vi "Equal Type Comparison.vi"(6 "verbose? (F)":bool, 8 "error in (no error)":errorcluster, 9 "Actual":variant, 10 "Expected":variant) -> (0 "error out":errorcluster, 2 "Equal Types?":bool, 3 "Verbose output":string)   [LabVIEW 2013, in "Caraya.lvlib" / "Assert.lvclass"]
uses:
  classes/Assert/Assert.lvclass
  <vilib>/Utility/VariantDataType/Type.ctl
  <vilib>/Utility/VariantDataType/VariantType.lvlib
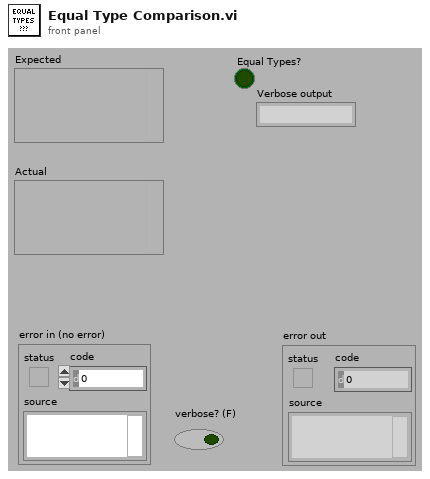
[diagram p1: front panel]
types:
  T1 = typedef "VariantType.lvlib/Type.ctl" = enum8{"Invalid Type", "Void", "I8", "I16", "I32", "I64", "U8", "U16", "U32", "U64", "Single Float", "Double Float", "Extended Float", "Single Complex", "Double Complex", "Extended Complex", "Enum U8", "Enum U16", "Enum U32", "Enum U64", "Single Float With Unit", "Double Float With Unit", "Extended Float With Unit", "Single Complex with Unit", "Double Complex with Unit", "Extended Complex with Unit", "Boolean", "String", "Path", "Picture", "Tag", "Array", "Cluster", "Variant", "LV Variant", "Waveform", "Timestamp", "Digital Waveform", "Digital Data", "ExpressData", "Refnum", "External Data", "VI", "Poly VI", "LabVIEW Class Instance", "Fixed Point"}
  T2 = typedef "VariantType.lvlib/RefnumType.ctl" = enum16{"NotARefnum", "UnknownRefnum", "Generic", "Datalog", "ByteStream", "Device", "Occurence", "TCPNetConnection", "Auto", "Menu", "Imaq", "Hardware", "DataSocket", "Visa", "IVI", "UDPNetConnection", "Notifier", "Queue", "Irda", "EventReg", "DotNet", "UserEvent", "Callback", "UNUSED_EMPTY_POSITION", "BlueToothNetConnection", "LVObjApp", "LVObjVI", "LVObjUnknown", "GenericClass", "UserDefinedRefnumTag", "DataValue", "RT FIFO", "TDMS File"}
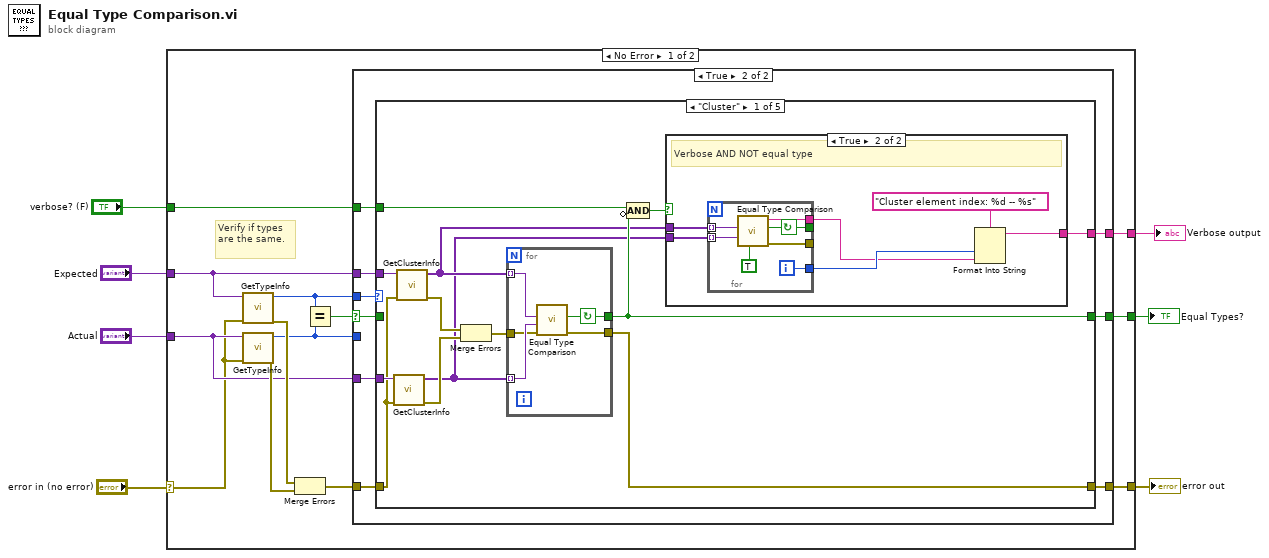
[diagram p0: block diagram]
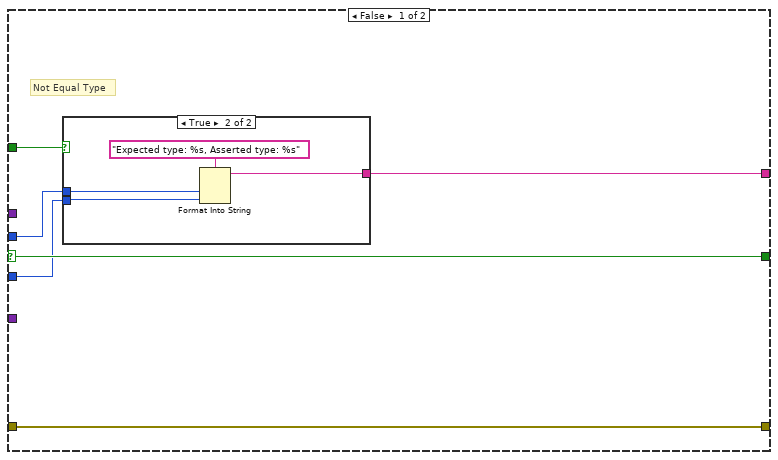
[diagram p2: hidden frame]
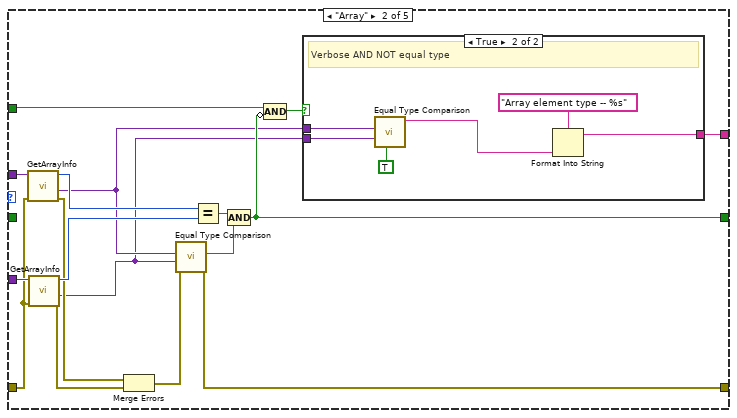
[diagram p5: hidden frame]
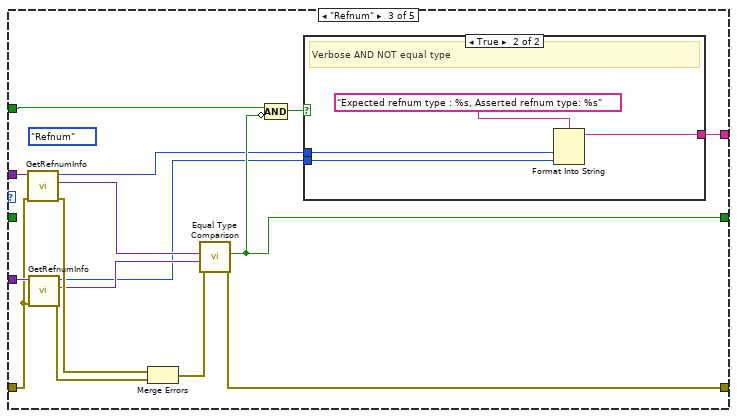
[diagram p7: hidden frame]
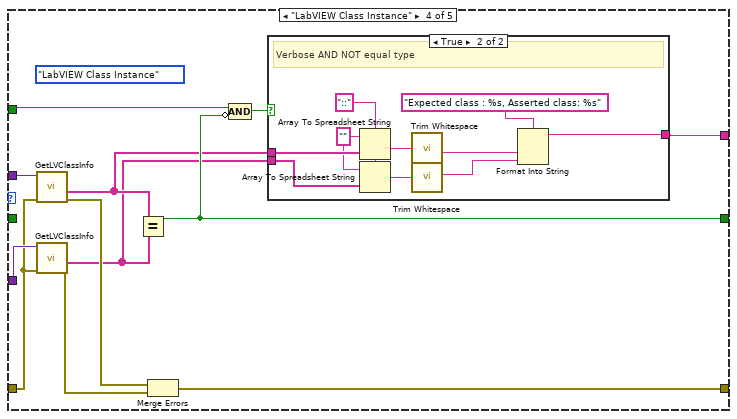
[diagram p9: hidden frame]
diagram:
  n1 = case shown="No Error" "error in (no error)" {
    selector: "error in (no error)" -> [w8 w137]
    tunnel: "Expected" -> [w15 _]
    tunnel: "Actual" -> [w14 _]
    tunnel: [w13 w137] -> w5
    tunnel: [w12 _] -> w4
    tunnel: "verbose? (F)" -> [w10 _]
    tunnel: [w9 _] -> w2
    frame No Error {
      # "Verify if types are the same."
      n2 = call <vilib>:"GetTypeInfo.vi"("error in (no error)"=w8, "Variant"=w15) -> ("error out"=w20:errorcluster, "Type Enum"=w17:T1)  [unwired: 5 in, 3 out]
      n3 = call <vilib>:"GetTypeInfo.vi"("error in (no error)"=w8, "Variant"=w14) -> ("error out"=w19:errorcluster, "Type Enum"=w11:T1)  [unwired: 5 in, 3 out]
      n4 = Merge Errors(w20, w19) -> (w16:errorcluster)
      n5 = Equal?(x=w17, y=w11) -> (x = y?=w18:bool)
      n6 = case shown="True" w18 {
        selector: w18 -> [w26 w38]
        tunnel: [w26 w37] -> w12
        tunnel: w17 -> [w24 w39]
        tunnel: w15 -> [_ w36]
        tunnel: w14 -> [_ w35]
        tunnel: w16 -> [w25 w34]
        tunnel: [w25 w33] -> w13
        tunnel: w11 -> [w22 _]
        tunnel: w10 -> [w23 w32]
        tunnel: [w21 w31] -> w9
        frame False {
          # "Not Equal Type"
          n7 = case shown="True" w23 {
            tunnel: w24 -> [_ w30]
            tunnel: w22 -> [_ w29]
            tunnel: [_ w27] -> w21
            frame False {
            }
            frame True {
              n8 = Format Into String(format string="Expected type: %s, Asserted type: %s", w30, w29) -> (resulting string=w27:string)  [unwired: 2 in, 1 out]
            }
          }
        }
        frame True {
          n9 = case shown="\"Cluster\"" w39 {
            tunnel: [w43 w73 w98 w115 w136] -> w37
            tunnel: w38 -> [_ _ _ _ w136]
            tunnel: w36 -> [w52 w87 w106 w124 _]
            tunnel: w35 -> [w51 w86 w104 w123 _]
            tunnel: w34 -> [w50 w82 w102 w122 w135]
            tunnel: [w49 w77 w107 w120 w135] -> w33
            tunnel: w32 -> [w45 w74 w99 w116 _]
            tunnel: [w40 w76 w100 w117 _] -> w31
            frame "Cluster" {
              n10 = call <vilib>:"GetClusterInfo.vi"("error in (no error)"=w50, "Variant"=w51) -> ("error out"=w46:errorcluster, "Cluster Elements"=w41:variant[])  [unwired: 8 in]
              n11 = call <vilib>:"GetClusterInfo.vi"("error in (no error)"=w50, "Variant"=w52) -> ("error out"=w47:errorcluster, "Cluster Elements"=w42:variant[])  [unwired: 8 in]
              n12 = Merge Errors(w47, w46) -> (w48:errorcluster)
              n13 = for {
                tunnel: [w68] -> w43
                tunnel: w42 -> [w70] mode=indexing
                tunnel: w41 -> [w69] mode=indexing
                tunnel: w48 -> [w67]
                tunnel: [w66] -> w49
                stop <- w68 continue-if-true
                n14 = call "Equal Type Comparison.vi"("error in (no error)"=w67, "Actual"=w69, "Expected"=w70) -> ("error out"=w66:errorcluster, "Equal Types?"=w68:bool)  [unwired: 6 in, 1 out]
              }
              n15 = Compound Arithmetic op=AND(w45, invert w43) -> (w44:bool)
              n16 = case shown="True" w44 {
                tunnel: w42 -> [_ w58]
                tunnel: w41 -> [_ w57]
                tunnel: [_ w56] -> w40
                frame False {
                }
                frame True {
                  # "Verbose AND NOT equal type"
                  n17 = for {
                    tunnel: [w63] -> _
                    tunnel: w58 -> [w65] mode=indexing
                    tunnel: w57 -> [w64] mode=indexing
                    tunnel: [w62] -> _
                    tunnel: [w60] -> w55
                    tunnel: [w59] -> w54
                    i -> [w60]
                    stop <- w63 continue-if-true
                    n18 = call "Equal Type Comparison.vi"("verbose? (F)"=TRUE, "Actual"=w64, "Expected"=w65) -> ("error out"=w62:errorcluster, "Equal Types?"=w63:bool, "Verbose output"=w59:string)  [unwired: 6 in]
                  }
                  n19 = Format Into String(format string="Cluster element index: %d -- %s", w55, w54) -> (resulting string=w56:string)  [unwired: 2 in, 1 out]
                }
              }
            }
            frame "Array" {
              n20 = call <vilib>:"GetArrayInfo.vi"("error in (no error)"=w82, "Variant"=w87) -> ("error out"=w81:errorcluster, "ArrayElement"=w72:variant, "NDims"=w85:i32)  [unwired: 6 in, 1 out]
              n21 = call <vilib>:"GetArrayInfo.vi"("error in (no error)"=w82, "Variant"=w86) -> ("error out"=w80:errorcluster, "ArrayElement"=w71:variant, "NDims"=w84:i32)  [unwired: 6 in, 1 out]
              n22 = Merge Errors(w81, w80) -> (w78:errorcluster)
              n23 = call "Equal Type Comparison.vi"("error in (no error)"=w78, "Actual"=w71, "Expected"=w72) -> ("error out"=w77:errorcluster, "Equal Types?"=w79:bool)  [unwired: 6 in, 1 out]
              n24 = Equal?(x=w85, y=w84) -> (x = y?=w83:bool)
              n25 = Compound Arithmetic op=AND(w83, w79) -> (w73:bool)
              n26 = Compound Arithmetic op=AND(w74, invert w73) -> (w75:bool)
              n27 = case shown="True" w75 {
                tunnel: w72 -> [_ w93]
                tunnel: w71 -> [_ w92]
                tunnel: [_ w91] -> w76
                frame False {
                }
                frame True {
                  # "Verbose AND NOT equal type"
                  n28 = call "Equal Type Comparison.vi"("verbose? (F)"=TRUE, "Actual"=w92, "Expected"=w93) -> ("Verbose output"=w90:string)  [unwired: 6 in, 2 out]
                  n29 = Format Into String(format string="Array element type -- %s", w90) -> (resulting string=w91:string)  [unwired: 2 in, 1 out]
                }
              }
            }
            frame "Refnum" {
              (unwired) Type."Refnum" ("Type Enum")
              n30 = call <vilib>:"GetRefnumInfo.vi"("error in (no error)"=w102, "Variant"=w106) -> ("error out"=w105:errorcluster, "StrictType"=w97:variant, "ReferenceType"=w95:T2)  [unwired: 6 in, 1 out]
              n31 = call <vilib>:"GetRefnumInfo.vi"("error in (no error)"=w102, "Variant"=w104) -> ("error out"=w103:errorcluster, "StrictType"=w96:variant, "ReferenceType"=w94:T2)  [unwired: 6 in, 1 out]
              n32 = Merge Errors(w105, w103) -> (w108:errorcluster)
              n33 = call "Equal Type Comparison.vi"("error in (no error)"=w108, "Actual"=w96, "Expected"=w97) -> ("error out"=w107:errorcluster, "Equal Types?"=w98:bool)  [unwired: 6 in, 1 out]
              n34 = Compound Arithmetic op=AND(w99, invert w98) -> (w101:bool)
              n35 = case shown="True" w101 {
                tunnel: [_ w112] -> w100
                tunnel: w95 -> [_ w110]
                tunnel: w94 -> [_ w109]
                frame False {
                }
                frame True {
                  # "Verbose AND NOT equal type"
                  n36 = Format Into String(format string="Expected refnum type : %s, Asserted refnum type: %s", w110, w109) -> (resulting string=w112:string)  [unwired: 2 in, 1 out]
                }
              }
            }
            frame "LabVIEW Class Instance" {
              (unwired) Type."LabVIEW Class Instance" ("Type Enum")
              n37 = call <vilib>:"GetLVClassInfo.vi"("error in (no error)"=w122, "Variant"=w124) -> ("error out"=w119:errorcluster, "Fully Qualified LV Class Name"=w114:string[])  [unwired: 7 in, 1 out]
              n38 = call <vilib>:"GetLVClassInfo.vi"("error in (no error)"=w122, "Variant"=w123) -> ("error out"=w121:errorcluster, "Fully Qualified LV Class Name"=w113:string[])  [unwired: 7 in, 1 out]
              n39 = Equal?(x=w114, y=w113) -> (x = y?=w115:bool)
              n40 = Merge Errors(w119, w121) -> (w120:errorcluster)
              n41 = Compound Arithmetic op=AND(w116, invert w115) -> (w118:bool)
              n42 = case shown="True" w118 {
                tunnel: [_ w134] -> w117
                tunnel: w114 -> [_ w131]
                tunnel: w113 -> [_ w133]
                frame False {
                }
                frame True {
                  w125 = "::" ("delimiter (Tab)")
                  w126 = "" ("format string")
                  # "Verbose AND NOT equal type"
                  n43 = Array To Spreadsheet String(delimiter (Tab)=w125, array=w131, 3:w126) -> (spreadsheet string=w130:string)
                  n44 = Array To Spreadsheet String(delimiter (Tab)=w125, array=w133, 3:w126) -> (spreadsheet string=w129:string)
                  n45 = call <vilib>:"Trim Whitespace.vi"("string"=w130) -> ("trimmed string"=w128:string)  [unwired: 1 in]
                  n46 = call <vilib>:"Trim Whitespace.vi"("string"=w129) -> ("trimmed string"=w127:string)  [unwired: 1 in]
                  n47 = Format Into String(format string="Expected class : %s, Asserted class: %s", w128, w127) -> (resulting string=w134:string)  [unwired: 2 in, 1 out]
                }
              }
            }
            frame Default {
            }
          }
        }
      }
    }
    frame Error {
    }
  }
  "Equal Types?" <- w4
  "error out" <- w5
  "Verbose output" <- w2
